vi "Determine Sector Edge Location.vi"(11 "Preanalysis Stage":bool) -> (2 "Left Sector Edge":u8, 3 "Right Sector Edge":u8)   [LabVIEW 2013]
doc: "Takes the average sector intensities and compares each average to the threshold value to determine which sector the edge is located in."
uses:
  Globals/Accumulated Sector Intensity.vi
  Globals/Sector Parameter Global.vi
  <vilib>/rvi/FIFO/Fifo_Resource/nirvififoEmulationReadFpgaImpl.vi
  <vilib>/rvi/DataTransferAndStorage/Container/Common/niFpgaContainerGetUniqueNameForEmu.vi
  <vilib>/rvi/interface/RandomDataEmulation/nirviRandomDataFPGAFIFO.vi
  <vilib>/rvi/interface/RandomDataEmulation/niFpgaRandomDataHandleErrors.vi
  <vilib>/rvi/DataTransferAndStorage/Container/XNode/niFpgaContainer.xnode
  <vilib>/rvi/FIFO/Fifo_Resource/nirvififoEmulationRead.vi
  <vilib>/rvi/interface/RandomDataEmulation/nirviRandomDataFpgaReadWriteTemplate.vi
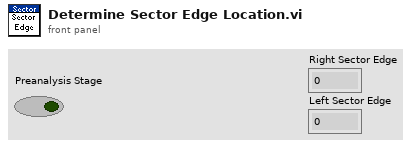
[diagram p1: front panel]
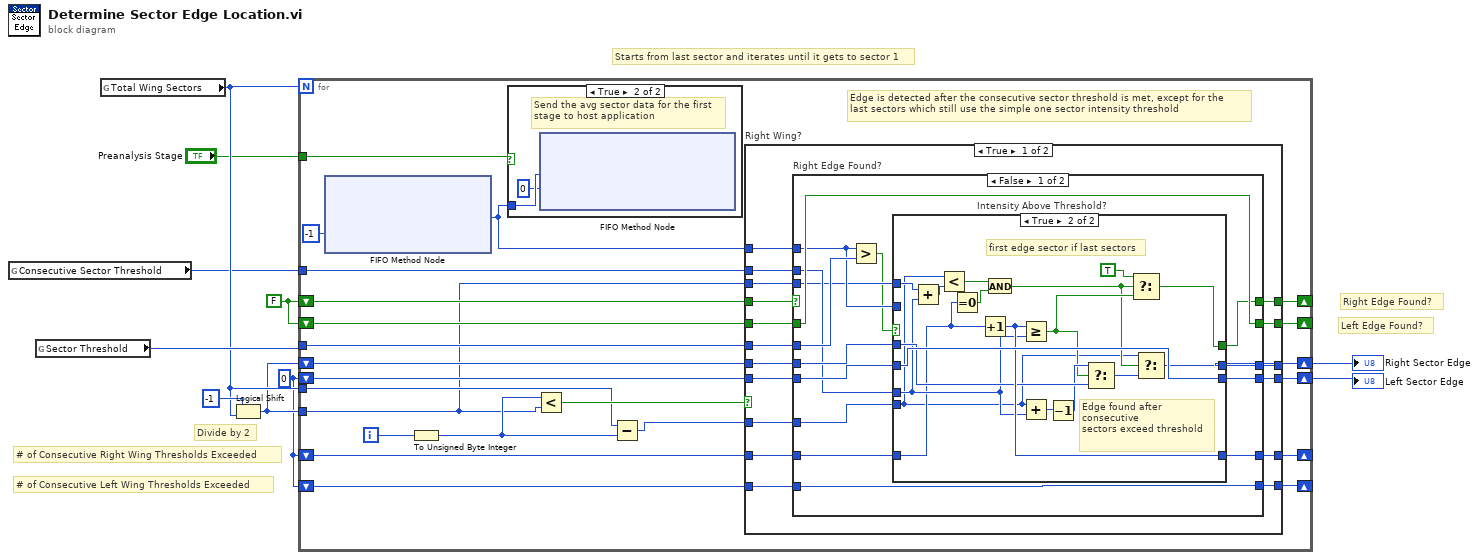
[diagram p0: block diagram]
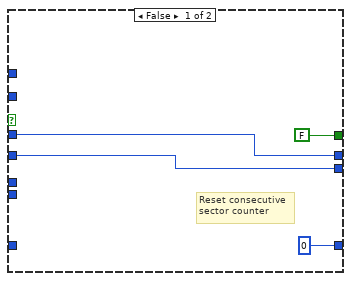
[diagram p3: hidden frame]
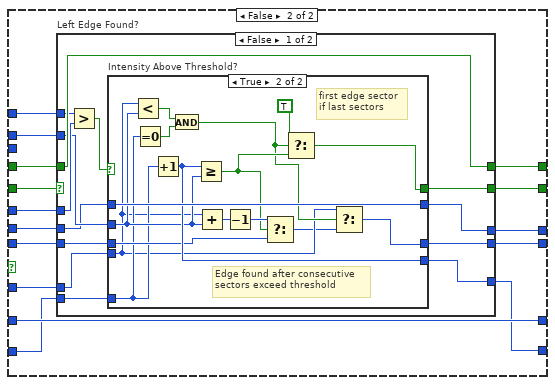
[diagram p5: hidden frame]
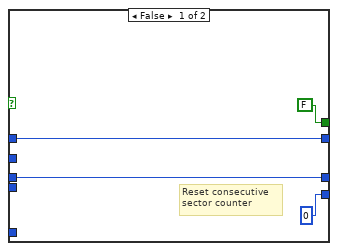
[diagram p6: hidden frame]
diagram:
  w2 = u8 0 ("Total Wing Sectors")
  w7 = FALSE ("Left Edge Found?")
  # "# of Consecutive Left Wing Thresholds Exceeded"
  # "# of Consecutive Right Wing Thresholds Exceeded"
  # "Starts from last sector and iterates until it gets to sector 1"
  # "Left Edge Found?"
  # "Right Edge Found?"
  # "Divide by 2"
  n1 = global read "Sector Parameter Global.vi" "Consecutive Sector Threshold"() -> (w1:u8)
  n2 = global read "Sector Parameter Global.vi" "Sector Threshold"() -> (w6:u8)
  n3 = global read "Accumulated Sector Intensity.vi" "Total Wing Sectors"() -> (w5:u8)
  n4 = Logical Shift(y=i16 -1, x=w5) -> (x << y=w3:u8)
  n5 = for {
    N: w5 -> [_]
    tunnel: w6 -> [w32]
    tunnel: w3 -> [w11]
    shift-right: [w30] -> _
    shift-left: w7 -> [w31]
    shift-right: [w23] -> _
    shift-left: w7 -> [w24]
    shift-right: [w28] -> w10
    shift-left: w3 -> [w27]
    shift-right: [w26] -> w9
    shift-left: w2 -> [w25]
    tunnel: w5 -> [w20]
    tunnel: "Preanalysis Stage" -> [w17]
    shift-right: [w14] -> _
    shift-left: w2 -> [w16]
    shift-right: [w13] -> _
    shift-left: w2 -> [w12]
    tunnel: w1 -> [w15]
    i -> [w29]
    # "Edge is detected after the consecutive sector threshold is met, except for the\nlast sectors which still use the simple one sector intensity threshold"
    n6 = xnode ("FIFO Method Node")("Timeout"=-1) -> ("Element"=w22:u8)  [unwired: 1 in, 2 out]
    n7 = To Unsigned Byte Integer(number=w29) -> (unsigned 8bit integer=w19:u8)
    n8 = case shown="True" w17 {
      tunnel: w22 -> [_ w35]
      frame False {
      }
      frame True {
        # "Send the avg sector data for the first\nstage to host application"
        n9 = xnode ("FIFO Method Node")("Element"=w35, "Timeout"=0) -> ()  [unwired: 1 in, 2 out]
      }
    }
    n10 = Less?(x=w19, y=w11) -> (x < y?=w33:bool)
    n11 = Subtract(x=w20, y=w19) -> (x-y=w18:u8)
    n12 = case "Right Wing?" shown="True" w33 {
      tunnel: w22 -> [w51 w110]
      tunnel: w32 -> [w50 w109]
      tunnel: w31 -> [w52 w101]
      tunnel: [w49 w108] -> w30
      tunnel: w18 -> [w48 w107]
      tunnel: [w47 w106] -> w28
      tunnel: w27 -> [w46 w105]
      tunnel: [w45 w104] -> w26
      tunnel: w25 -> [w44 w103]
      tunnel: w24 -> [w43 w102]
      tunnel: [w42 w100] -> w23
      tunnel: w16 -> [w41 w99]
      tunnel: w15 -> [w40 w96]
      tunnel: [w39 w99] -> w14
      tunnel: [w38 w97] -> w13
      tunnel: w12 -> [w37 w98]
      tunnel: w11 -> [w36 _]
      frame True {
        n13 = case "Right Edge Found?" shown="False" w52 {
          selector: w52 -> [_ w92]
          tunnel: w51 -> [w61 _]
          tunnel: w50 -> [w67 _]
          tunnel: [w59 w92] -> w49
          tunnel: w48 -> [w56 _]
          tunnel: [w66 w95] -> w47
          tunnel: w46 -> [w65 w95]
          tunnel: [w64 w94] -> w45
          tunnel: w44 -> [w63 w94]
          tunnel: w43 -> [w62 w93]
          tunnel: [w62 w93] -> w42
          tunnel: w41 -> [w60 w91]
          tunnel: w40 -> [w55 _]
          tunnel: [w58 w91] -> w39
          tunnel: [w57 w90] -> w38
          tunnel: w37 -> [w57 w90]
          tunnel: w36 -> [w54 _]
          frame False {
            n14 = Greater?(x=w61, y=w67) -> (0:w53:bool)
            n15 = case "Intensity Above Threshold?" shown="True" w53 {
              tunnel: w56 -> [_ w73]
              tunnel: [w71 w74] -> w66
              tunnel: w65 -> [w71 w87]
              tunnel: [w70 w89] -> w64
              tunnel: w63 -> [w70 w89]
              tunnel: w61 -> [_ _]
              tunnel: w60 -> [_ w77]
              tunnel: w55 -> [_ w84]
              tunnel: [FALSE w80] -> w59
              tunnel: [u8 0 w88] -> w58
              tunnel: w54 -> [_ w82]
              frame False {
                # "Reset consecutive\nsector counter"
              }
              frame True {
                # "Edge found after consecutive\nsectors exceed threshold"
                # "first edge sector if last sectors"
                n16 = Add(x=w82, y=w84) -> (x+y=w83:u8)
                n17 = Less?(x=w73, y=w83) -> (x < y?=w79:bool)
                n18 = Equal To 0?(x=w77) -> (x = 0?=w78:bool)
                n19 = Increment(x=w77) -> (x+1=w88:u8)
                n20 = And(x=w79, y=w78) -> (x .and. y?=w76:bool)
                n21 = Greater Or Equal?(x=w88, y=w84) -> (x >= y?=w81:bool)
                n22 = Add(x=w73, y=w84) -> (x+y=w86:u8)
                n23 = Decrement(x=w86) -> (x-1=w85:u8)
                n24 = Select(t=w85, s=w81, f=w87) -> (s? t:f=w75:u8)
                n25 = Select(t=TRUE, s=w76, f=w81) -> (s? t:f=w80:bool)
                n26 = Select(t=w73, s=w76, f=w75) -> (s? t:f=w74:u8)
              }
            }
          }
          frame True {
          }
        }
      }
      frame False {
        n27 = case "Left Edge Found?" shown="False" w102 {
          selector: w102 -> [_ w145]
          tunnel: w110 -> [w121 _]
          tunnel: w109 -> [w123 _]
          tunnel: [w122 w146] -> w108
          tunnel: w107 -> [w114 _]
          tunnel: [w111 w148] -> w106
          tunnel: w105 -> [w112 w148]
          tunnel: [w116 w147] -> w104
          tunnel: w103 -> [w115 w147]
          tunnel: w101 -> [w122 w146]
          tunnel: [w118 w145] -> w100
          tunnel: w98 -> [w119 w144]
          tunnel: [w117 w144] -> w97
          tunnel: w96 -> [w113 _]
          frame False {
            n28 = Greater?(x=w121, y=w123) -> (0:w120:bool)
            n29 = case "Intensity Above Threshold?" shown="True" w120 {
              tunnel: w114 -> [_ w130]
              tunnel: [w127 w129] -> w116
              tunnel: w115 -> [w127 w141]
              tunnel: [w126 w143] -> w111
              tunnel: w112 -> [w126 w143]
              tunnel: w119 -> [_ w137]
              tunnel: w113 -> [_ w138]
              tunnel: [FALSE w133] -> w118
              tunnel: [u8 0 w142] -> w117
              frame False {
                # "Reset consecutive\nsector counter"
              }
              frame True {
                # "Edge found after consecutive\nsectors exceed threshold"
                # "first edge sector \nif last sectors"
                n30 = Less?(x=w130, y=w138) -> (x < y?=w136:bool)
                n31 = Equal To 0?(x=w137) -> (x = 0?=w135:bool)
                n32 = Increment(x=w137) -> (x+1=w142:u8)
                n33 = And(x=w136, y=w135) -> (x .and. y?=w131:bool)
                n34 = Greater Or Equal?(x=w142, y=w138) -> (x >= y?=w134:bool)
                n35 = Add(x=w130, y=w138) -> (x+y=w140:u8)
                n36 = Decrement(x=w140) -> (x-1=w139:u8)
                n37 = Select(t=w139, s=w134, f=w141) -> (s? t:f=w128:u8)
                n38 = Select(t=TRUE, s=w131, f=w134) -> (s? t:f=w133:bool)
                n39 = Select(t=w130, s=w131, f=w128) -> (s? t:f=w129:u8)
              }
            }
          }
          frame True {
          }
        }
      }
    }
  }
  "Right Sector Edge" <- w10
  "Left Sector Edge" <- w9
